vi "Test Parse Amount.vi"() -> ()   [LabVIEW 2026]
doc: "Caraya unit test for Parse Amount.vi, generated by lvai_generate_test.\n\nOne static subVI call per case. Every assertion takes its error in from Define Test rather than from the assertion before it, so a failing case cannot stop a later one - chaining them silently loses cases, measured.\n\nThe error cluster carries the FIRST failure only. Read the JUnit report for all of them."
uses:
  <vilib>/addons/_JKI Toolkits/Caraya/classes/Test/Test.lvclass
  <vilib>/addons/_JKI Toolkits/Caraya/classes/Assert/Assert.lvclass
panel:
  out "error out":errorcluster
  in  "error in":errorcluster
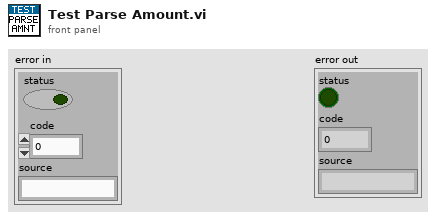
[diagram p1: front panel]
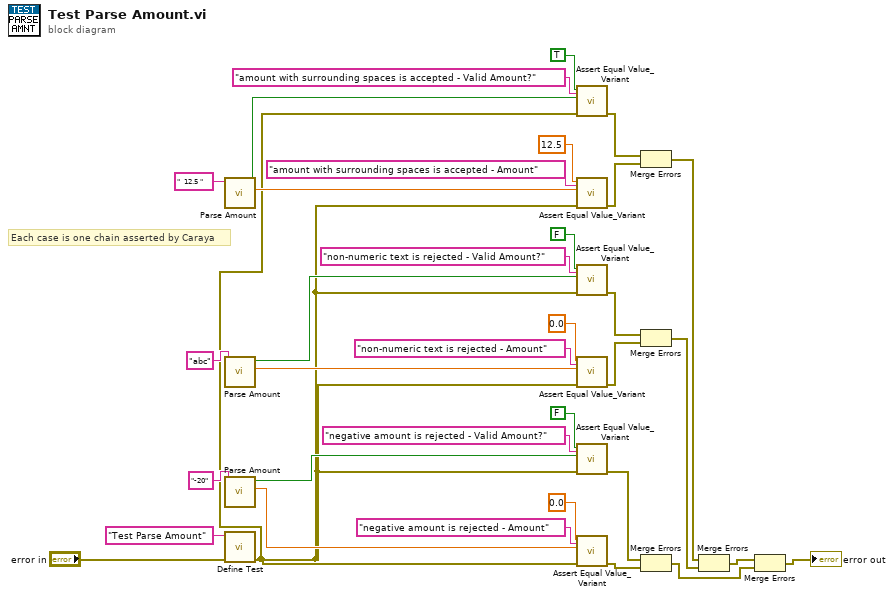
[diagram p0: block diagram]
diagram:
  # "Each case is one chain asserted by Caraya"
  n1 = call "Parse Amount.vi"("User Input"="  12.5 ") -> ("Amount"=w6:dbl, "Valid Amount?"=w5:bool)  [unwired: 8 in, 1 out]
  n2 = call "Parse Amount.vi"("User Input"="abc") -> ("Amount"=w15:dbl, "Valid Amount?"=w14:bool)  [unwired: 8 in, 1 out]
  n3 = call "Parse Amount.vi"("User Input"="-20") -> ("Amount"=w24:dbl, "Valid Amount?"=w23:bool)  [unwired: 8 in, 1 out]
  n4 = call <vilib>:"Define Test.vi"("error in (no error)"="error in", "Label (VI Title)"="Test Parse Amount") -> ("error out"=w3:errorcluster)  [unwired: 8 in, 1 out]
  n5 = call <vilib>:"Assert Equal Value_Variant.vi"("Label"="amount with surrounding spaces is accepted - Valid Amount?", "error in (no error)"=w3, "Actual"=w5, "Expected"=TRUE ("expected 1")) -> ("error out"=w9:errorcluster)  [unwired: 6 in, 1 out]
  n6 = call <vilib>:"Assert Equal Value_Variant.vi"("Label"="amount with surrounding spaces is accepted - Amount", "error in (no error)"=w3, "Actual"=w6, "Expected"=12.5 ("expected 2")) -> ("error out"=w12:errorcluster)  [unwired: 6 in, 1 out]
  n7 = call <vilib>:"Assert Equal Value_Variant.vi"("Label"="non-numeric text is rejected - Valid Amount?", "error in (no error)"=w3, "Actual"=w14, "Expected"=FALSE ("expected 3")) -> ("error out"=w18:errorcluster)  [unwired: 6 in, 1 out]
  n8 = call <vilib>:"Assert Equal Value_Variant.vi"("Label"="non-numeric text is rejected - Amount", "error in (no error)"=w3, "Actual"=w15, "Expected"=0.0 ("expected 4")) -> ("error out"=w21:errorcluster)  [unwired: 6 in, 1 out]
  n9 = call <vilib>:"Assert Equal Value_Variant.vi"("Label"="negative amount is rejected - Valid Amount?", "error in (no error)"=w3, "Actual"=w23, "Expected"=FALSE ("expected 5")) -> ("error out"=w27:errorcluster)  [unwired: 6 in, 1 out]
  n10 = call <vilib>:"Assert Equal Value_Variant.vi"("Label"="negative amount is rejected - Amount", "error in (no error)"=w3, "Actual"=w24, "Expected"=0.0 ("expected 6")) -> ("error out"=w30:errorcluster)  [unwired: 6 in, 1 out]
  n11 = Merge Errors(w9, w12) -> (w31:errorcluster)
  n12 = Merge Errors(w18, w21) -> (w32:errorcluster)
  n13 = Merge Errors(w27, w30) -> (w33:errorcluster)
  n14 = Merge Errors(w31, w32) -> (w34:errorcluster)
  n15 = Merge Errors(w34, w33) -> (→"error out":errorcluster)
